vi "Globals.vi"() -> ()   [LabVIEW 2026]
uses:
  Typedefs/ServoCommand.ctl
  Typedefs/BeltCtrl.ctl
  Typedefs/System_State.ctl
panel:
  out "Last Image Frame":string
  in  "System State":T1 items=["Idle", "Classify", "Sort"]
  in  "MotorCtrl":T2
  out "Auto":bool
  out "Throughput (obj/min)":dbl
  out "ClrCount 4":i32
  out "ClrCount 3":i32
  out "ClrCount 2":i32
  out "ClrCount 1":i32
  out "ClrGate 4":bool
  out "ClrGate 3":bool
  out "ClrGate 2":bool
  out "ClrGate 1":bool
  out "Camera Feed":T3(plugin-control)
  in  "Servo Command":T4
  in  "Stop System":bool
  in  "Motor Speed (%)":dbl min=0.0 max=100.0
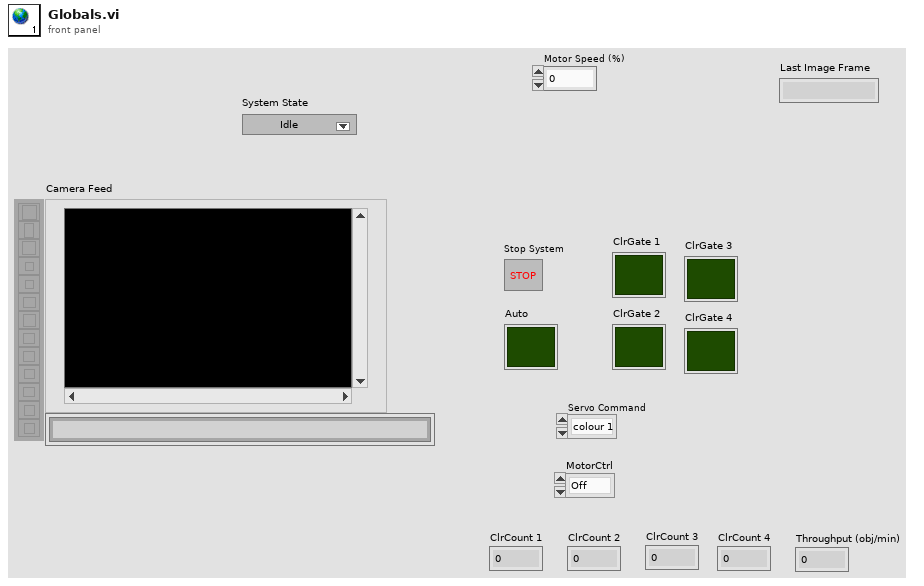
[diagram p1: front panel]
types:
  T1 = typedef "System_State.ctl" = u16
  T2 = typedef "BeltCtrl.ctl" = enum16{"Off", "Forward", "Back", "Coast", "Brake", ""}
  T3 = typedef "IMAQ Image.ctl" = refnum<image>
  T4 = typedef "ServoCommand.ctl" = enum16{"colour 1", "Colour2", "Colour3", "Reject"}
diagram:
